vi "numCmd_Recv_TwoDbl.vi"(7 "Command Name":string, 10 "Initial Value 2":dbl, 11 "Initial Value 1":dbl) -> (0 "error out":errorcluster, 1 "Any Changed":bool, 2 "Value 2":dbl, 3 "Value 1":dbl)   [LabVIEW 2019, in "Trajectory_Library.lvlib"]
uses:
  Trajectory_Library.lvlib
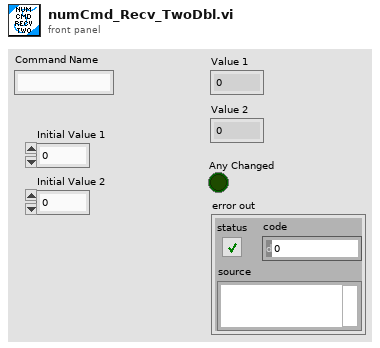
[diagram p1: front panel]
types:
  T1 = cluster{"Initial Value 1":dbl, "Initial Value 2":dbl}
  T2 = cluster{"Initial Value 1":bool, "Initial Value 2":bool}
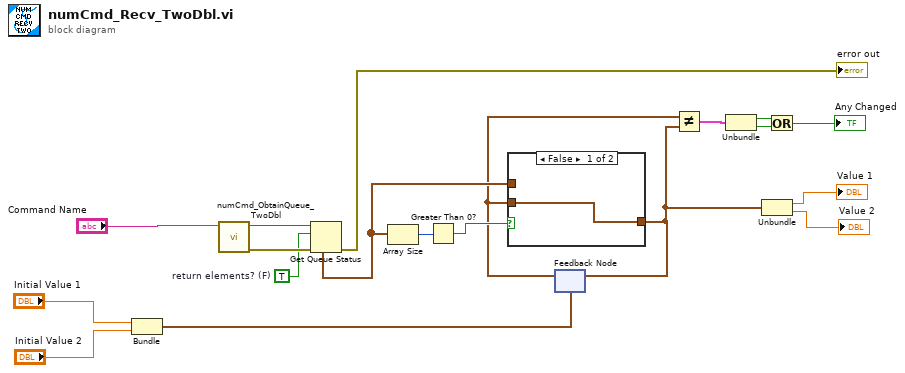
[diagram p0: block diagram]
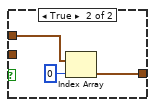
[diagram p2: hidden frame]
diagram:
  w9 = TRUE  # return elements? (F)
  n1 = Bundle("Initial Value 1"="Initial Value 1", "Initial Value 2"="Initial Value 2") -> (w7:T1)  [unwired: 1 in]
  n2 = call "numCmd_ObtainQueue_TwoDbl.vi"("Command Name"="Command Name") -> ("error out"=w14:errorcluster, "queue out"=w15:refnum<queue>)  [unwired: 9 in]
  n3 = Get Queue Status(queue=w15, return elements? (F)=w9, error in (no error)=w14) -> (error out=→"error out":errorcluster, elements=w11:cluster{dbl, dbl}[])  [unwired: 6 out]
  n4 = Array Size(array=w11) -> (size(s)=w13:i32)
  n5 = Greater Than 0?(x=w13) -> (x > 0?=w12:bool)
  n6 = feedback #1(w7) -> (w10:T1)
  n7 = case shown="False" w12 {
    tunnel: w11 -> [_ w23]
    tunnel: [w20 w21] -> w1
    tunnel: w10 -> [w20 _]
    frame False {
    }
    frame True {
      n8 = Index Array(array=w23, index=0) -> (element=w21:cluster{dbl, dbl})
    }
  }
  n9 = feedback-in #1(w1) -> ()
  n10 = Not Equal?(x=w10, y=w1) -> (x != y?=w6:T2)
  n11 = Unbundle(w6) -> ("Initial Value 1"=w5:bool, "Initial Value 2"=w4:bool)
  n12 = Unbundle(w1) -> ("Initial Value 1"=→"Value 1":dbl, "Initial Value 2"=→"Value 2":dbl)
  n13 = Or(x=w5, y=w4) -> (x .or. y?=→"Any Changed":bool)
